vi "Curvature of Bezier Spline.vi"(11 "bezier spline waypts":T1) -> (3 "curvature":dbl[][](array[numeric]))   [LabVIEW 2020]
uses:
  Types/Bezier Spline.ctl
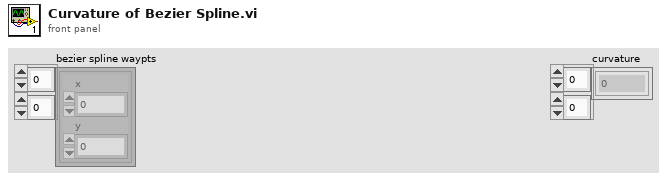
[diagram p1: front panel]
types:
  T1 = typedef "Bezier Spline.ctl" = cluster{"x":sgl, "y":sgl}[][]
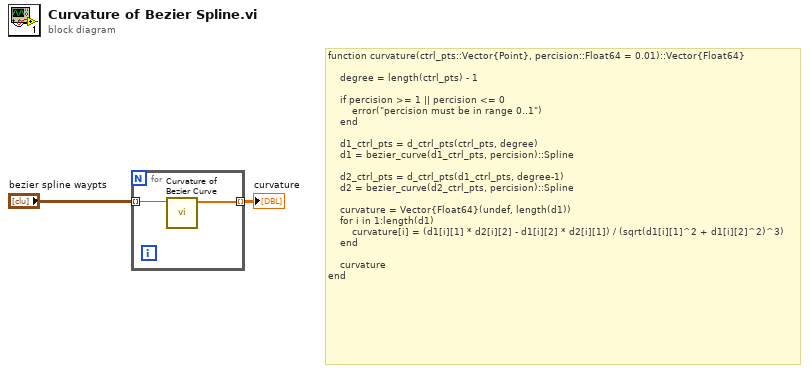
[diagram p0: block diagram]
diagram:
  # "function curvature(ctrl_pts::Vector{Point}, percision::Float64 = 0.01)::Vector{Float64}\n\n    degree = length(ctrl_pts) - 1\n\n    if percision >= 1 || percision <= 0\n        error(\"percision must be in range 0..1\")\n    end\n\n    d1_ctrl_pts = d_ctrl_pts(ctrl_pts, degree)\n    d1 = bezier_curve(d1_ctrl_pts, percision)::Spline\n\n    d2_ctrl_pts = d_ctrl_pts(d1_ctrl_pts, degree-1)\n    d2 = bezier_curve(d2_ctrl_pts, percision)::Spline\n\n    curvature = Vector{Float64}(undef, length(d1))\n    for i in 1:length(d1)\n        curvature[i] = (d1[i][1] * d2[i][2] - d1[i][2] * d2[i][1]) / (sqrt(d1[i][1]^2 + d1[i][2]^2)^3)\n    end\n\n    curvature\nend"
  n1 = for {
    tunnel: "bezier spline waypts" -> [w4] mode=indexing
    tunnel: [w3] -> w1 mode=indexing
    n2 = call "Curvature of Bezier Curve.vi"("curve"=w4) -> ("curvature"=w3:dbl[])  [unwired: 10 in]
  }
  "curvature" <- w1
